vi "String To Indexed Enum_csm.vi"(7 "Variant":variant, 8 "error in (no error)":errorcluster, 11 "String":string) -> (0 "error out":errorcluster, 3 "Enum":variant)   [LabVIEW 2017, in "API String Arguments Support.lvlib"]
doc: "Converts a string to an indexed enum type.\n\n\n> [!NOTE] <b>Indexed Enum</b>\n>\n> Format: `[Index Number][Separator][Enum String]`.\n>\n> The index number supports multiple numeric representations.\n>\n> Example of Index Number using `==` separator:\n> `1 == boolean | 2 == string | 4 == dbl | 8 == number`\n>\n> Example of Index Number using `--` separator:\n> `0x01 -- boolean | 0x02 -- string | 0x04 -- dbl | 0x08 -- number`\n>\n> Example of Index Number using `__` separator:\n> `0b0001 __ boolean | 0b0100 __ dbl | 0b1000 __ number`\n\n\n _<b>Conversion Rule 1: No Index Number</b>_\n\n Convert by string matching.\n\n Example Enum = {AAA, BBBB, CCCC}\n\n - String \"AAA\" converts to Enum(AAA), numeric value 0.\n - String \"CCC\" converts to Enum(CCC), numeric value 2.\n\n _<b>Conversion Rule 2: With Index Number</b>_\n\n Convert by either string matching or index number matching.\n\n Example Enum = {1- AAA, 5 - BBBB, 9 - CCCC}\n\n - String \"AAA\" converts to Enum(1- AAA), numeric value 0.\n - String \"5\" converts to Enum(5 - BBBB), numeric value 1.\n - String \"9 - CCCC\" converts to Enum(9 - CCCC), numeric value 2.\n\n-- <b>Controls</b> --\n- <b>String</b>: Input string.\n- <b>Enum Prototype</b>: Enum prototype.\n\n-- <b>Indicators</b> --\n- <b>Enum</b>: Converted enum value."
uses:
  API String Arguments Support.lvlib
  <userlib>/_NEVSTOP/Communicable State Machine(CSM)/Communicable State Machine.lvlib
  <userlib>/_NEVSTOP/Communicable State Machine(CSM)/_Shared/CSM Shared.lvlib
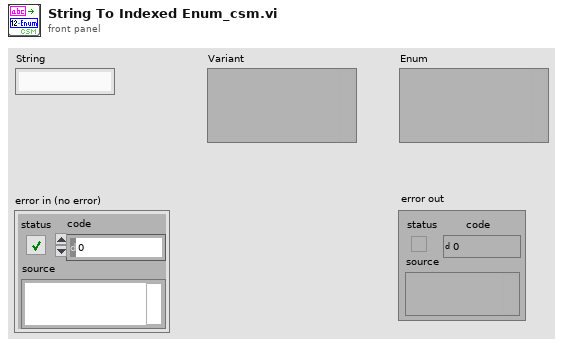
[diagram p1: front panel]
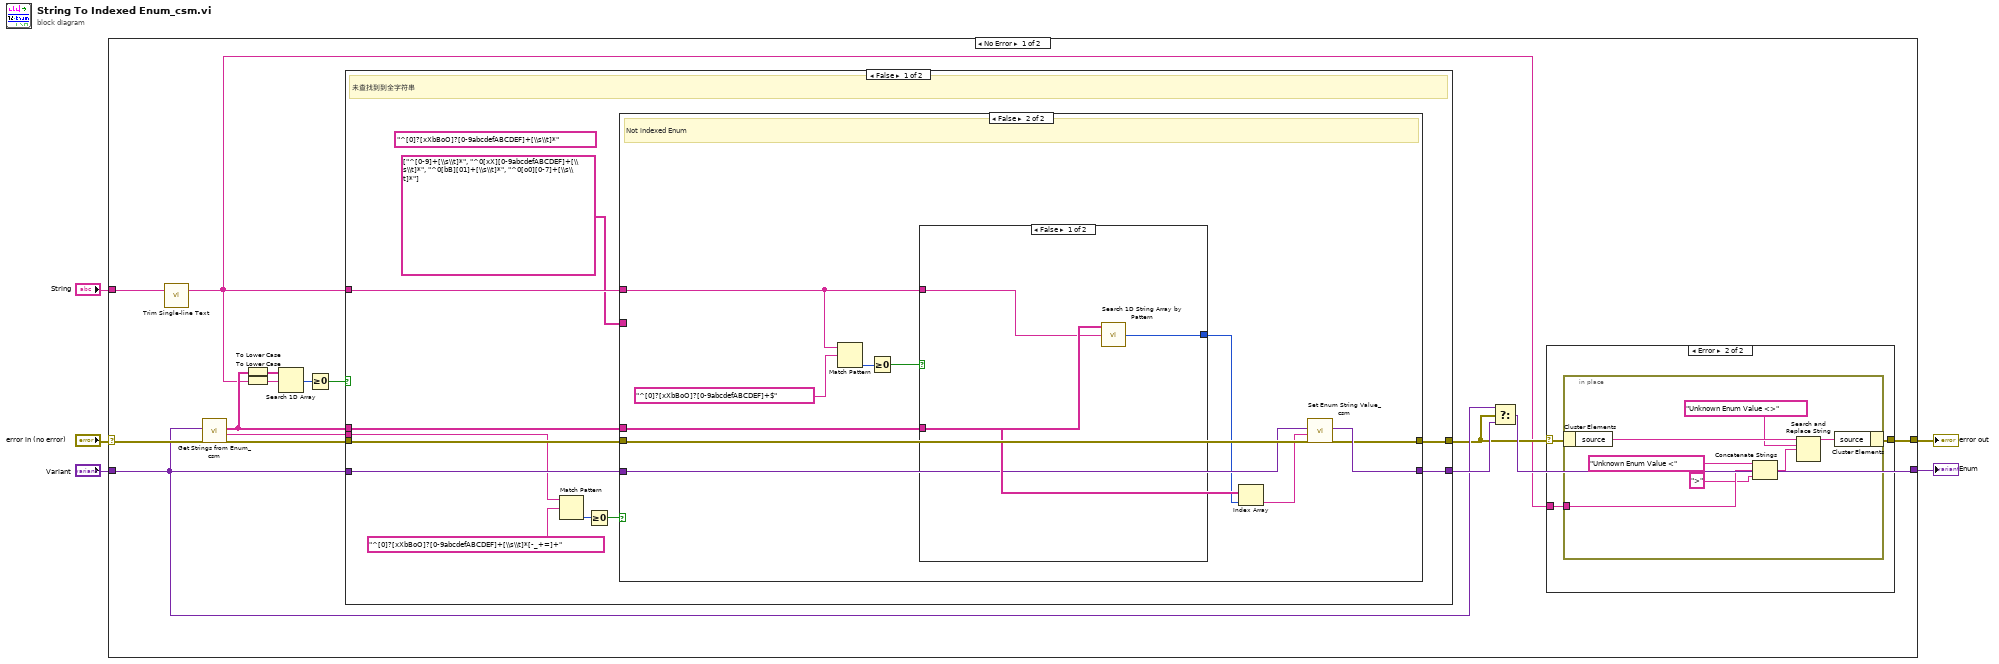
[diagram p0: block diagram]
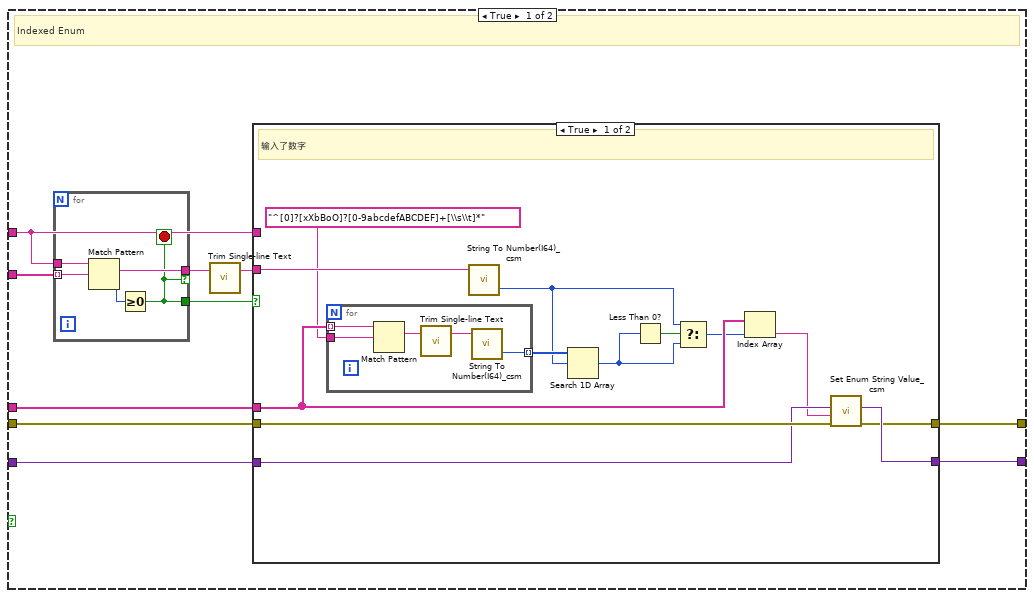
[diagram p3: hidden frame]
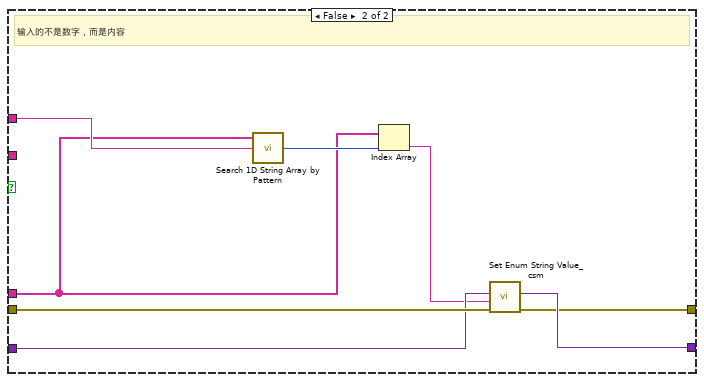
[diagram p4: hidden frame]
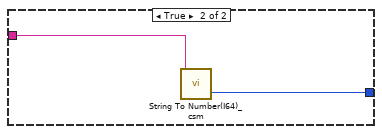
[diagram p5: hidden frame]
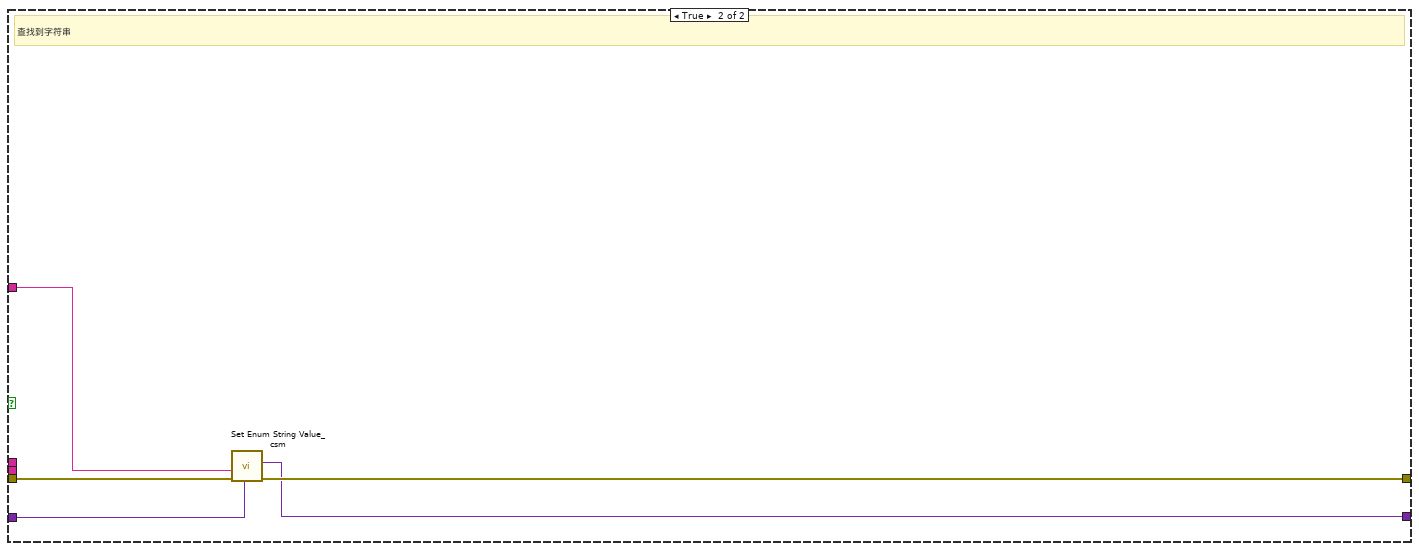
[diagram p6: hidden frame]
diagram:
  n1 = case shown="No Error" "error in (no error)" {
    selector: "error in (no error)" -> [w20 w106]
    tunnel: "Variant" -> [w17 w105]
    tunnel: "String" -> [w7 _]
    tunnel: [w16 w105] -> w2
    tunnel: [w8 w106] -> w1
    frame No Error {
      n2 = call <userlib>:"Trim Single-line Text.vi"("single-line text"=w7) -> ("trimed text"=w6:string)  [unwired: 2 in]
      n3 = call <userlib>:"Get Strings from Enum_csm.vi"("error in (no error)"=w20, "Enum"=w17) -> ("error out"=w19:errorcluster, "String Value"=w15:string, "Enum Strings"=w11:string[])  [unwired: 6 in, 1 out]
      n4 = To Lower Case(string=w11) -> (all lower case string=w12:string[])
      n5 = To Lower Case(string=w6) -> (all lower case string=w13:string)
      n6 = Search 1D Array(1D array=w12, element=w13) -> (index of element=w14:i32)  [unwired: 1 in]
      n7 = Greater Or Equal To 0?(x=w14) -> (x >= 0?=w10:bool)
      n8 = case shown="False" w10 {
        tunnel: w19 -> [w42 w104]
        tunnel: [w41 w100] -> w18
        tunnel: w17 -> [w40 w103]
        tunnel: [w39 w101] -> w9
        tunnel: w15 -> [w37 _]
        tunnel: w11 -> [w34 _]
        tunnel: w6 -> [w33 w102]
        frame False {
          (unwired) "^[0]?[xXbBoO]?[0-9abcdefABCDEF]+[\\s\\t]*" ("regular expression")
          # "未查找到到全字符串"
          n9 = Match Pattern(string=w37, regular expression="^[0]?[xXbBoO]?[0-9abcdefABCDEF]+[\\s\\t]*[-_+=]+") -> (offset past match=w38:i32)  [unwired: 1 in, 3 out]
          n10 = Greater Or Equal To 0?(x=w38) -> (x >= 0?=w35:bool)
          n11 = case shown="False" w35 {
            tunnel: w42 -> [w52 w94]
            tunnel: w34 -> [w48 w93]
            tunnel: w33 -> [w45 w86]
            tunnel: [w51 w92] -> w41
            tunnel: w40 -> [w50 w91]
            tunnel: [w49 w90] -> w39
            tunnel: string[] ["^[0-9]+[\\s\\t]*", "^0[xX][0-9abcdefABCDEF]+[\\s\\t]*", "^0[bB][01]+[\\s\\t]*", "^0[o0][0-7]+[\\s\\t]*"] -> [w44 _]
            frame True {
              # "Indexed Enum"
              n12 = for {
                tunnel: w44 -> [w53] mode=indexing
                tunnel: w45 -> [w57]
                tunnel: [w56] -> w47 if=w54
                tunnel: [w54] -> w43
                stop <- w54 stop-if-true
                n13 = Match Pattern(string=w57, regular expression=w53) -> (match substring=w56:string, offset past match=w55:i32)  [unwired: 1 in, 2 out]
                n14 = Greater Or Equal To 0?(x=w55) -> (x >= 0?=w54:bool)
              }
              n15 = call <userlib>:"Trim Single-line Text.vi"("single-line text"=w47) -> ("trimed text"=w46:string)  [unwired: 2 in]
              n16 = case shown="True" w43 {
                tunnel: [w70 w83] -> w51
                tunnel: w52 -> [w69 w82]
                tunnel: w50 -> [w68 w81]
                tunnel: [w67 w80] -> w49
                tunnel: w48 -> [w66 w76]
                tunnel: w45 -> [_ w78]
                tunnel: w46 -> [w65 _]
                frame True {
                  # "输入了数字"
                  n17 = for {
                    tunnel: w66 -> [w75] mode=indexing
                    tunnel: [w71] -> w63 mode=indexing
                    tunnel: "^[0]?[xXbBoO]?[0-9abcdefABCDEF]+[\\s\\t]*" ("regular expression") -> [w74]
                    n18 = Match Pattern(string=w75, regular expression=w74) -> (match substring=w73:string)  [unwired: 1 in, 3 out]
                    n19 = call <userlib>:"Trim Single-line Text.vi"("single-line text"=w73) -> ("trimed text"=w72:string)  [unwired: 2 in]
                    n20 = call "String To Number(I64)_csm.vi"("String"=w72) -> ("Numeric"=w71:u64)  [unwired: 4 in]
                  }
                  n21 = call "String To Number(I64)_csm.vi"("String"=w65) -> ("Numeric"=w60:u64)  [unwired: 4 in]
                  n22 = Search 1D Array(1D array=w63, element=w60) -> (index of element=w61:i32)  [unwired: 1 in]
                  n23 = Less Than 0?(x=w61) -> (x < 0?=w62:bool)
                  n24 = Select(t=w60, s=w62, f=w61) -> (s? t:f=w59:u64)
                  n25 = Index Array(array=w66, index=w59) -> (element=w64:string)
                  n26 = call <userlib>:"Set Enum String Value_csm.vi"("error in (no error)"=w69, "String Value"=w64, "Default Enum Value"=w68) -> ("error out"=w67:errorcluster, "Enum"=w70:variant)  [unwired: 7 in]
                }
                frame False {
                  # "输入的不是数字，而是内容"
                  n27 = call "Search 1D String Array by Pattern.vi"("Reg text"=w78, "1D String Array"=w76) -> ("index of element"=w77:i32)  [unwired: 3 in]
                  n28 = Index Array(array=w76, index=w77) -> (element=w79:string)
                  n29 = call <userlib>:"Set Enum String Value_csm.vi"("error in (no error)"=w82, "String Value"=w79, "Default Enum Value"=w81) -> ("error out"=w80:errorcluster, "Enum"=w83:variant)  [unwired: 7 in]
                }
              }
            }
            frame False {
              # "Not indexed Enum"
              n30 = Match Pattern(string=w86, regular expression="^[0]?[xXbBoO]?[0-9abcdefABCDEF]+$") -> (offset past match=w85:i32)  [unwired: 1 in, 3 out]
              n31 = Greater Or Equal To 0?(x=w85) -> (x >= 0?=w84:bool)
              n32 = case shown="False" w84 {
                tunnel: w93 -> [w97 _]
                tunnel: [w95 w98] -> w89
                tunnel: w86 -> [w96 w99]
                frame False {
                  n33 = call "Search 1D String Array by Pattern.vi"("Reg text"=w96, "1D String Array"=w97) -> ("index of element"=w95:i32)  [unwired: 3 in]
                }
                frame True {
                  n34 = call "String To Number(I64)_csm.vi"("String"=w99) -> ("Numeric"=w98:u64)  [unwired: 4 in]
                }
              }
              n35 = Index Array(array=w93, index=w89) -> (element=w88:string)
              n36 = call <userlib>:"Set Enum String Value_csm.vi"("error in (no error)"=w94, "String Value"=w88, "Default Enum Value"=w91) -> ("error out"=w90:errorcluster, "Enum"=w92:variant)  [unwired: 7 in]
            }
          }
        }
        frame True {
          # "查找到字符串"
          n37 = call <userlib>:"Set Enum String Value_csm.vi"("error in (no error)"=w104, "String Value"=w102, "Default Enum Value"=w103) -> ("error out"=w101:errorcluster, "Enum"=w100:variant)  [unwired: 7 in]
        }
      }
      n38 = Select(t=w17, s=w9, f=w18) -> (s? t:f=w16:variant)
      n39 = case shown="Error" w9 {
        selector: w9 -> [w21 w24]
        tunnel: [w21 w23] -> w8
        tunnel: w6 -> [_ w22]
        frame No Error {
        }
        frame Error {
          n40 = in-place {
            in-place-border: w22 -> [w27]
            n41 = in-place-cluster #1(w24) -> ("source"=w30:string)
            n42 = Concatenate Strings("Unknown Enum Value <" ("string"), w27, ">" ("string")) -> (w25:string)
            n43 = Search and Replace String(input string=w30, search string="Unknown Enum Value <>", replace string=w25) -> (result string=w31:string)  [unwired: 5 in, 3 out]
            n44 = in-place-cluster #1("source"=w31) -> (w23:errorcluster)
          }
        }
      }
    }
    frame Error {
    }
  }
  "Enum" <- w2
  "error out" <- w1
